vi "serial.vi"() -> ()   [LabVIEW 2017]
uses:
  <vilib>/Instr/_visa.llb/VISA Configure Serial Port (Instr).vi
panel:
  out "SUICHE":bool
  out "TEMPERATURA":dbl(slide) scale=0.0..100.0
  out "read buffer":string
  in  "PARAR":bool
  in  "PUERTO":refnum<visa-resource-name>="COM4"
  in  "Izquierda":bool
  in  "Derecha":bool
  in  "VELOCIDAD":dbl(knob) scale=0.0..100.0
  in  "LED2":bool
  in  "LED1":bool
  in  "stop":bool
  # "GIRO"
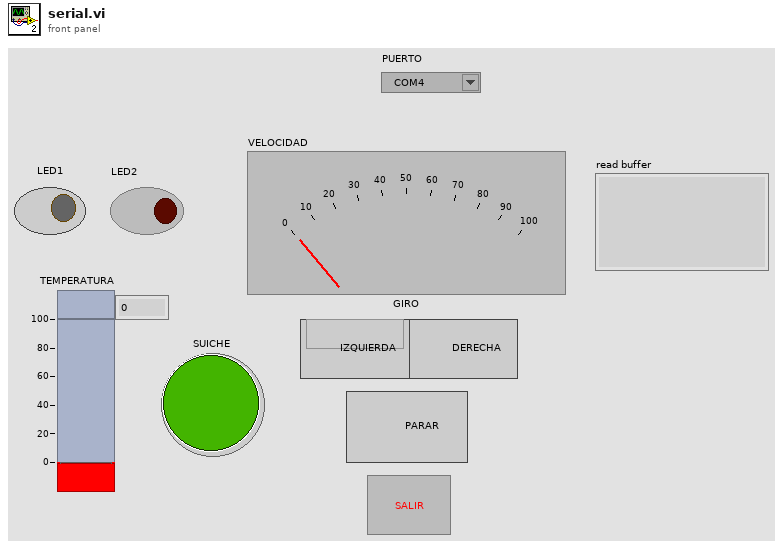
[diagram p1: front panel]
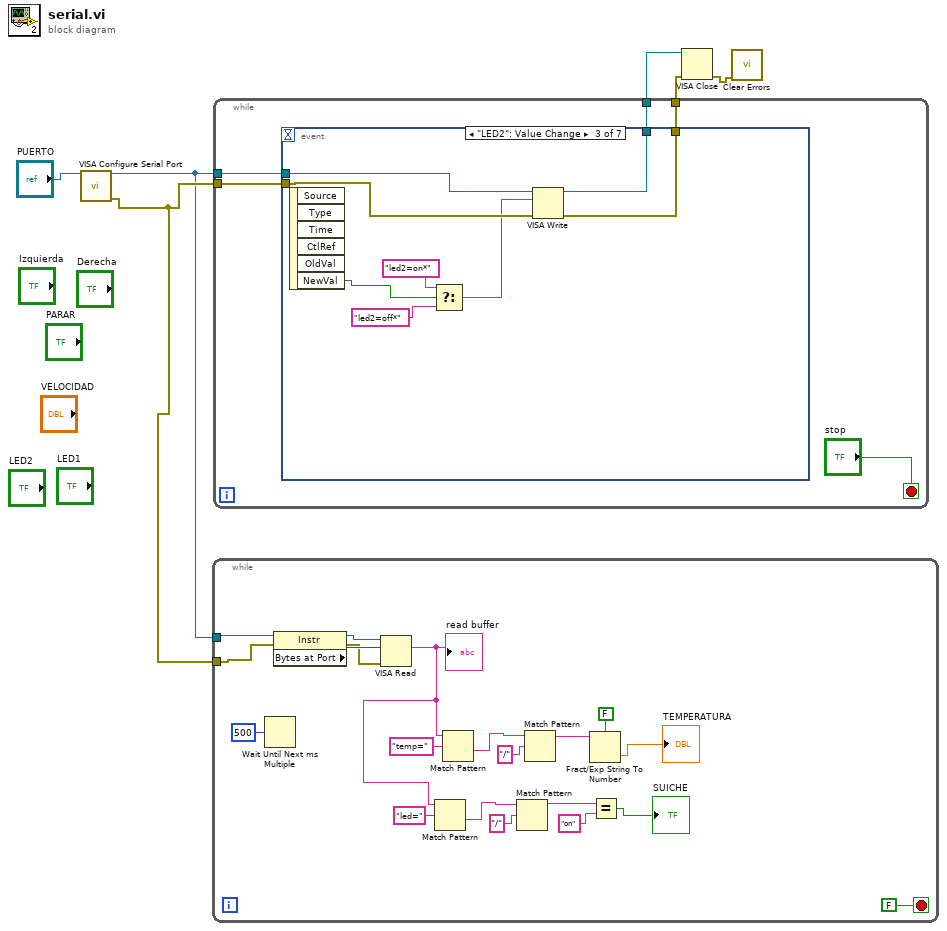
[diagram p0: block diagram]
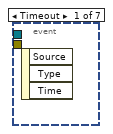
[diagram p2: hidden frame]
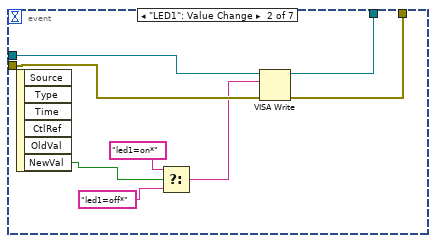
[diagram p3: hidden frame]
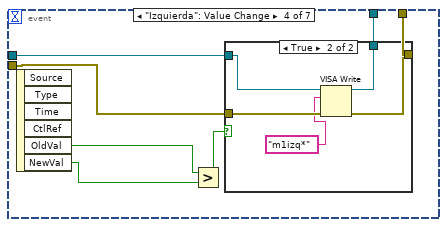
[diagram p4: hidden frame]
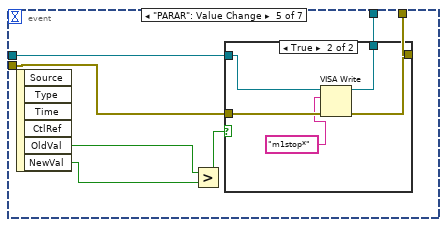
[diagram p6: hidden frame]
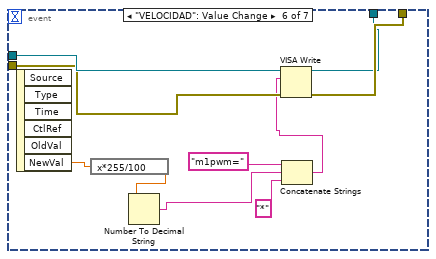
[diagram p8: hidden frame]
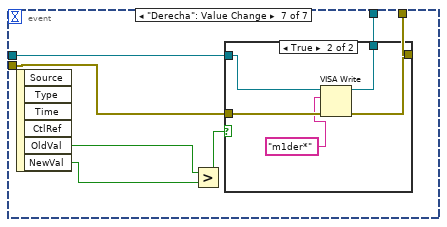
[diagram p9: hidden frame]
diagram:
  n1 = call-poly "VISA Configure Serial Port"("VISA resource name"="PUERTO") -> ("VISA resource name out"=w1:refnum<visa-resource-name>, "error out"=w2:errorcluster)  [unwired: 13 in]
  n2 = while {
    tunnel: w2 -> [w21]
    tunnel: w1 -> [w22]
    stop <- FALSE stop-if-true
    n3 = Wait Until Next ms Multiple(millisecond multiple=u32 500) -> ()  [unwired: 1 out]
    n4 = property class="Instr"(reference=w22, error in=w21) -> (reference out=w24:refnum<visa-resource-name>, error out=w23:errorcluster, "Bytes at Port"=w25:u32)
    n5 = VISA Read(VISA resource name=w24, byte count=w25, error in (no error)=w23) -> (read buffer=w8:string)  [unwired: 3 out]
    "read buffer" <- w8
    n6 = Match Pattern(string=w8, regular expression="led=") -> (after substring=w12:string)  [unwired: 1 in, 3 out]
    n7 = Match Pattern(string=w8, regular expression="temp=") -> (after substring=w18:string)  [unwired: 1 in, 3 out]
    n8 = Match Pattern(string=w12, regular expression="/") -> (before substring=w10:string)  [unwired: 1 in, 3 out]
    n9 = Match Pattern(string=w18, regular expression="/") -> (before substring=w16:string)  [unwired: 1 in, 3 out]
    n10 = Fract/Exp String To Number(use system decimal point (T)=FALSE, string=w16) -> (number=→"TEMPERATURA":dbl)  [unwired: 2 in, 1 out]
    n11 = Equal?(x=w10, y="on") -> (x = y?=→"SUICHE":bool)
  }
  n12 = while {
    tunnel: w1 -> [w30]
    tunnel: w2 -> [w29]
    tunnel: [w28] -> w5
    tunnel: [w27] -> w4
    stop <- "stop" stop-if-true
    n13 = event shown="[2] \"LED2\": Value Change" {
      selector: _ -> [_ _ _ _ _ _ _]
      dyn-events: _ -> [_ _ _ _ _ _ _]
      timeout: _ -> [_ _ _ _ _ _ _]
      tunnel: w30 -> [_ w39 w47 w54 w66 w81 w88]
      tunnel: w29 -> [_ w38 w46 w53 w65 w80 w87]
      tunnel: [_ w33 w41 w52 w64 w78 w86] -> w28
      tunnel: [_ w32 w40 w51 w63 w79 w85] -> w27
      event Timeout {
        n14 = event-data() -> ()  [unwired: 1 in, 3 out]
      }
      event "LED1": Value Change {
        n15 = event-data() -> ("NewVal"=w37:bool)  [unwired: 1 in, 5 out]
        n16 = Select(t="led1=on*", s=w37, f="led1=off*") -> (s? t:f=w34:string)
        n17 = VISA Write(VISA resource name=w39, write buffer=w34, error in (no error)=w38) -> (VISA resource name out=w33:refnum<visa-resource-name>, error out=w32:errorcluster)  [unwired: 1 out]
      }
      event "LED2": Value Change {
        n18 = event-data() -> ("NewVal"=w45:bool)  [unwired: 1 in, 5 out]
        n19 = Select(t="led2=on*", s=w45, f="led2=off*") -> (s? t:f=w42:string)
        n20 = VISA Write(VISA resource name=w47, write buffer=w42, error in (no error)=w46) -> (VISA resource name out=w41:refnum<visa-resource-name>, error out=w40:errorcluster)  [unwired: 1 out]
      }
      event "Izquierda": Value Change {
        n21 = event-data() -> ("OldVal"=w50:bool, "NewVal"=w49:bool)  [unwired: 1 in, 4 out]
        n22 = Greater?(x=w50, y=w49) -> (0:w48:bool)
        n23 = case shown="True" w48 {
          tunnel: w54 -> [_ w59]
          tunnel: w53 -> [_ w58]
          tunnel: [_ w57] -> w52
          tunnel: [_ w56] -> w51
          frame False {
          }
          frame True {
            n24 = VISA Write(VISA resource name=w59, write buffer="m1izq*", error in (no error)=w58) -> (VISA resource name out=w57:refnum<visa-resource-name>, error out=w56:errorcluster)  [unwired: 1 out]
          }
        }
      }
      event "PARAR": Value Change {
        n25 = event-data() -> ("OldVal"=w62:bool, "NewVal"=w61:bool)  [unwired: 1 in, 4 out]
        n26 = Greater?(x=w62, y=w61) -> (0:w60:bool)
        n27 = case shown="True" w60 {
          tunnel: w66 -> [_ w71]
          tunnel: w65 -> [_ w70]
          tunnel: [_ w69] -> w64
          tunnel: [_ w68] -> w63
          frame False {
          }
          frame True {
            n28 = VISA Write(VISA resource name=w71, write buffer="m1stop*", error in (no error)=w70) -> (VISA resource name out=w69:refnum<visa-resource-name>, error out=w68:errorcluster)  [unwired: 1 out]
          }
        }
      }
      event "VELOCIDAD": Value Change {
        n29 = event-data() -> ("NewVal"=w73:dbl)  [unwired: 1 in, 5 out]
        n30 = expression code="x*255/100"(w73) -> (w72:dbl)
        n31 = Number To Decimal String(number=w72) -> (decimal integer string=w76:string)  [unwired: 1 in]
        n32 = Concatenate Strings("m1pwm=" ("string"), w76, "*" ("string")) -> (w74:string)
        n33 = VISA Write(VISA resource name=w81, write buffer=w74, error in (no error)=w80) -> (VISA resource name out=w78:refnum<visa-resource-name>, error out=w79:errorcluster)  [unwired: 1 out]
      }
      event "Derecha": Value Change {
        n34 = event-data() -> ("OldVal"=w84:bool, "NewVal"=w83:bool)  [unwired: 1 in, 4 out]
        n35 = Greater?(x=w84, y=w83) -> (0:w82:bool)
        n36 = case shown="True" w82 {
          tunnel: w88 -> [_ w93]
          tunnel: w87 -> [_ w92]
          tunnel: [_ w91] -> w86
          tunnel: [_ w90] -> w85
          frame False {
          }
          frame True {
            n37 = VISA Write(VISA resource name=w93, write buffer="m1der*", error in (no error)=w92) -> (VISA resource name out=w91:refnum<visa-resource-name>, error out=w90:errorcluster)  [unwired: 1 out]
          }
        }
      }
    }
  }
  n38 = VISA Close(VISA resource name=w5, error in (no error)=w4) -> (error out=w3:errorcluster)
  n39 = call <vilib>:"Clear Errors.vi"("error in (no error)"=w3) -> ()  [unwired: 5 in, 2 out]
